vi "ReadFile.vi"(8 "error in (no error)":errorcluster, 11 "object in":refnum<class "ChannelManagerUI.lvclass">) -> (0 "error out":errorcluster, 3 "object out":refnum<class "ChannelManagerUI.lvclass">)   [LabVIEW 2021, in "Channel.lvlib" / "ChannelManagerUI.lvlib" / "ChannelManagerUI.lvclass"]
doc: "Reads the channels File"
uses:
  ChannelManagerUI.lvclass
  ChannelsManager/ChannelsManager/ChannelsManager.lvclass
  ChannelManagerUI.lvclass/ChannelManagerUI.ctl
panel:
  out "Channel Names":string[](array[string])
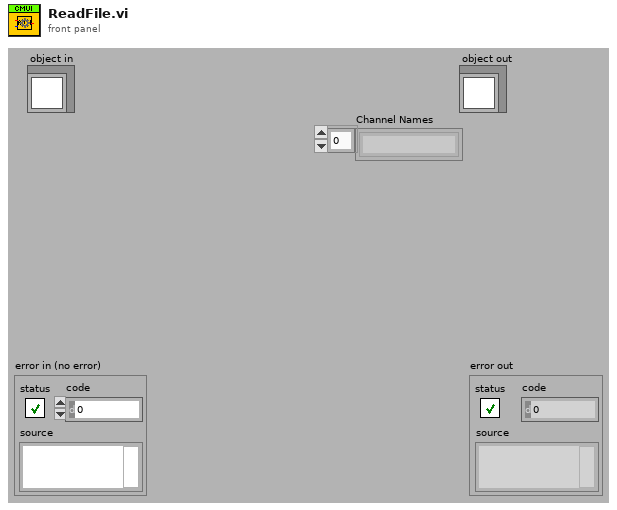
[diagram p1: front panel]
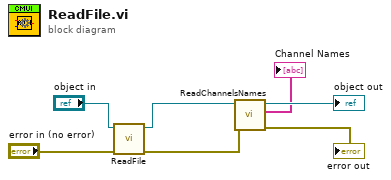
[diagram p0: block diagram]
diagram:
  n1 = call-parent "ReadFile.vi"("error in (no error)"="error in (no error)", "object in"="object in") -> ("error out"=w1:errorcluster, "object out"=w7:refnum<class "ChannelManagerUI.lvclass">)  [unwired: 8 in]
  n2 = call-dynamic "ReadChannelsNames.vi"("error in (no error)"=w1, "ChannelManagerUI in"=w7) -> ("error out"=→"error out":errorcluster, "Channel Names"=→"Channel Names":string[], "ChannelManagerUI out"=→"object out":refnum<class "ChannelManagerUI.lvclass">)  [unwired: 7 in]
